vi "Set Ann Slope.vi"(8 "error in":errorcluster, 9 "Active Plot":u32, 10 "Points":cluster{"X":dbl, "Y":dbl}[](array[cluster]), 11 "XY Plot":refnum<vi>) -> (0 "error out":errorcluster, 3 "XY Plot out":refnum<vi>)   [LabVIEW 2025, in "XY Plotter.lvlib" / "XY Plotter.lvclass"]
uses:
  XY Plotter.lvclass
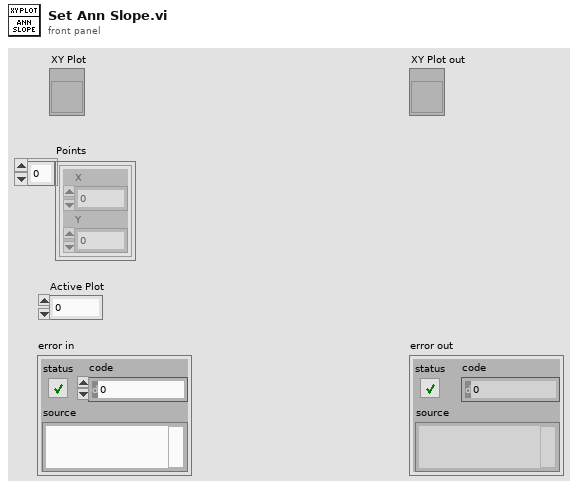
[diagram p1: front panel]
types:
  T1 = cluster{"Name":string, "Color":u32, "Style":u8, "Point Style":u8, "Name Visible":bool, "Allow Drag":bool, "Annotation Mode":u32, "Plot":i32, "Index":i32, "Position":cluster{"X":dbl, "Y":dbl}, "X Scale":u32, "Y Scale":u32, "Show Arrow":bool, "Lock Name":bool, "Plot Area":i32, "Label Offset":cluster{"X":dbl, "Y":dbl}}
  T2 = typedef "LVAnnotationListTypeDef.ctl" = cluster{"Name":string, "Color":u32, "Style":u8, "Point Style":u8, "Name Visible":bool, "Allow Drag":bool, "Annotation Mode":u32, "Plot":i32, "Index":i32, "Position":cluster{"X":dbl, "Y":dbl}, "X Scale":u32, "Y Scale":u32, "Show Arrow":bool, "Lock Name":bool, "Plot Area":i32, "Label Offset":cluster{"X":dbl, "Y":dbl}}[]
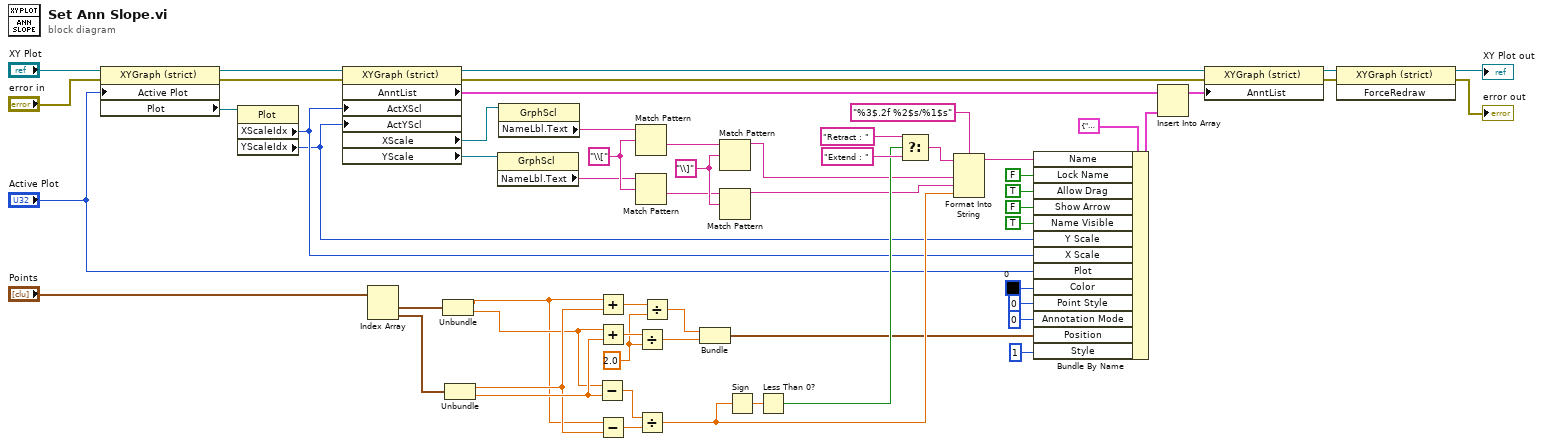
[diagram p0: block diagram]
diagram:
  w23 = 2.0 ("y")
  w42 = "\\]" ("regular expression")
  w43 = "\\[" ("regular expression")
  n1 = property class="XYGraph (strict)"(reference="XY Plot", error in="error in", "Active Plot"="Active Plot") -> (reference out=w52:refnum<vi>, error out=w50:errorcluster, "Plot"=w47:refnum<vi>)
  n2 = property class="Plot"(reference=w47) -> ("XScaleIdx"=w7:u32, "YScaleIdx"=w6:u32)  [unwired: 1 in, 2 out]
  n3 = property class="XYGraph (strict)"(reference=w52, error in=w50, "ActXScl"=w7, "ActYScl"=w6) -> (reference out=w51:refnum<vi>, error out=w49:errorcluster, "AnntList"=w53:T2, "XScale"=w45:refnum<vi>, "YScale"=w44:refnum<vi>)
  n4 = Index Array(array="Points") -> (element #1=w36:cluster{"X":dbl, "Y":dbl}, element #2=w37:cluster{"X":dbl, "Y":dbl})  [unwired: 2 in]
  n5 = Unbundle(w36) -> ("X"=w32:dbl, "Y"=w33:dbl)
  n6 = Unbundle(w37) -> ("X"=w34:dbl, "Y"=w35:dbl)
  n7 = property class="GrphScl"(reference=w44) -> ("NameLbl.Text"=w38:string)  [unwired: 1 in, 2 out]
  n8 = property class="GrphScl"(reference=w45) -> ("NameLbl.Text"=w39:string)  [unwired: 1 in, 2 out]
  n9 = Subtract(x=w33, y=w35) -> (x-y=w21:dbl)
  n10 = Add(x=w32, y=w34) -> (x+y=w22:dbl)
  n11 = Add(x=w33, y=w35) -> (x+y=w24:dbl)
  n12 = Subtract(x=w32, y=w34) -> (x-y=w20:dbl)
  n13 = Match Pattern(string=w39, regular expression=w43) -> (after substring=w40:string)  [unwired: 1 in, 3 out]
  n14 = Match Pattern(string=w38, regular expression=w43) -> (after substring=w41:string)  [unwired: 1 in, 3 out]
  n15 = Divide(x=w24, y=w23) -> (x/y=w26:dbl)
  n16 = Divide(x=w21, y=w20) -> (x/y=w15:dbl)
  n17 = Divide(x=w22, y=w23) -> (x/y=w25:dbl)
  n18 = Bundle(w25, w26) -> (w9:cluster{dbl, dbl})  [unwired: 1 in]
  n19 = Match Pattern(string=w40, regular expression=w42) -> (before substring=w17:string)  [unwired: 1 in, 3 out]
  n20 = Match Pattern(string=w41, regular expression=w42) -> (before substring=w16:string)  [unwired: 1 in, 3 out]
  n21 = Sign(1:w15) -> (0:w27:dbl)
  n22 = Less Than 0?(x=w27) -> (x < 0?=w28:bool)
  n23 = Select(t="Retract : " ("format string"), s=w28, f="Extend : " ("format string")) -> (s? t:f=w31:string)
  n24 = Format Into String(format string="%3$.2f %2$s/%1$s", initial string=w31, w17, w16, w15) -> (resulting string=w11:string)  [unwired: 1 in, 1 out]
  n25 = Bundle By Name(cluster=T1 {"Name"="", "Color"=0, "Style"=0, "Point Style"=0, "Name Visible"=FALSE, "Allow Drag"=FALSE, "Annotation Mode"=0, "Plot"=0, "Index"=0, "Position"={"X"=0.0, "Y"=0.0}, "X Scale"=0, "Y Scale"=0, "Show Arrow"=FALSE, "Lock Name"=FALSE, "Plot Area"=0, "Label Offset"={"X"=0.0, "Y"=0.0}} ("new element/subarray"), "Name"=w11, "Lock Name"=FALSE, "Allow Drag"=TRUE, "Show Arrow"=FALSE, "Name Visible"=TRUE, "Y Scale"=w6, "X Scale"=w7, "Plot"="Active Plot", "Color"=u32 0, "Point Style"=u8 0, "Annotation Mode"=u32 0, "Position"=w9, "Style"=u8 1) -> (w54:T1)
  n26 = Insert Into Array(array=w53, new element=w54) -> (w59:T2)  [unwired: 1 in]
  n27 = property class="XYGraph (strict)"(reference=w51, error in=w49, "AnntList"=w59) -> (reference out=w2:refnum<vi>, error out=w57:errorcluster)
  n28 = invoke class="XYGraph (strict)" method="ForceRedraw"(reference=w2, error in=w57) -> (reference out=→"XY Plot out":refnum<vi>, error out=→"error out":errorcluster)  [unwired: 1 in, 1 out]
